vi "Manage error.vi"(8 "error in":errorcluster, 11 "Error":refnum<queue>) -> (0 "error out":errorcluster)   [LabVIEW 2021]
uses:
  Type defs/Message cluster.ctl
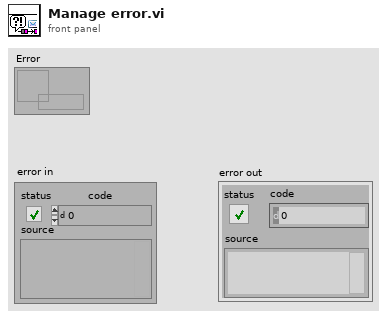
[diagram p1: front panel]
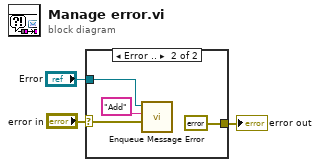
[diagram p0: block diagram]
diagram:
  n1 = case shown="Error .." "error in" {
    selector: "error in" -> [w4 w8]
    tunnel: [w4 errorcluster {"status"=FALSE, "code"=0, "source"=""} ("error IO")] -> w2
    tunnel: "Error" -> [_ w5]
    frame No Error {
    }
    frame Error {
      n2 = call "Enqueue Message Error.vi"("Data"=w8, "Message"="Add", "queue in"=w5) -> ()  [unwired: 7 in, 2 out]
    }
  }
  "error out" <- w2
